vi "Own20261012_GetFormulaParameterInfo.vi"() -> ()   [LabVIEW 2024]
panel:
  out "error out":errorcluster caption="错误输出"
  out "terminal_id":refnum<vi>
  out "is_input":bool
  out "name":string
  in  "parameter_id":u32
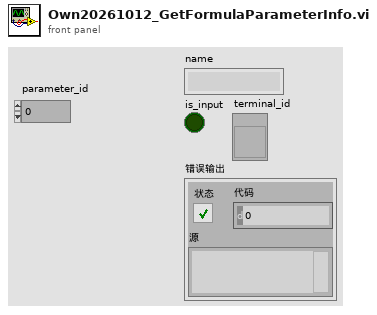
[diagram p1: front panel]
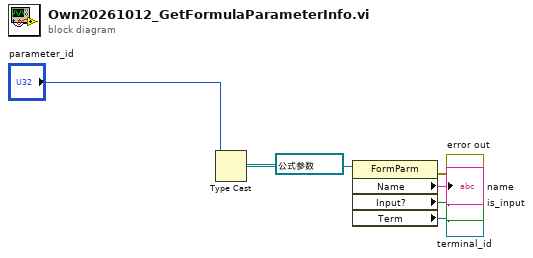
[diagram p0: block diagram]
diagram:
  n1 = Type Cast(type=refnum<vi> refnum ("引用"), x="parameter_id") -> (*(type *) &x=w5:refnum<vi>)
  n2 = property class="FormParm"(reference=w5) -> (error out=→"error out":errorcluster, "Name"=→"name":string, "Input?"=→"is_input":bool, "Term"=→"terminal_id":refnum<vi>)  [unwired: 1 in, 1 out]
